vi "OverlayCross.vi"(4 "Color":u32(colorbox)=16711680, 6 "Angle":dbl, 7 "GroupName":string, 8 "error in":errorcluster, 9 "Size":i32=10, 10 "Point":T1, 11 "Image Reference In":T2) -> (0 "error out":errorcluster, 3 "Image Reference Out":T2)   [LabVIEW 2020, in "OpenLvVision_Overlays.lvlib"]
doc: "Overlay a arc on top of an image."
uses:
  OpenLvVision_Overlays.lvlib
  <vilib>/OpenLvVision/OpenLvVision_Image/Management/TypeDef/OLV Image.ctl
  TypeDefs/PointI32.ctl
  <vilib>/OpenLvVision/OpenLvVision_Image/Management/OLV Management.lvlib
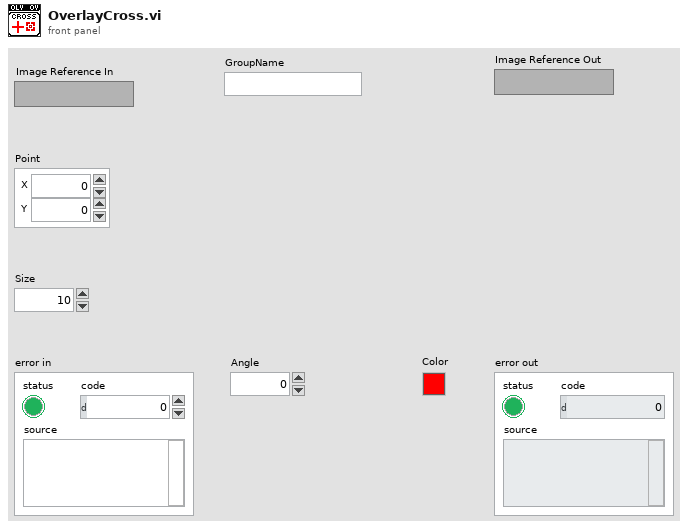
[diagram p1: front panel]
types:
  T1 = typedef "OpenLvVision_Overlays.lvlib/PointI32.ctl" = cluster{"X":i32, "Y":i32}
  T2 = typedef "OLV OpenLvVision_Image.lvlib/OLV Management.lvlib/OLV Image.ctl" = refnum<image>
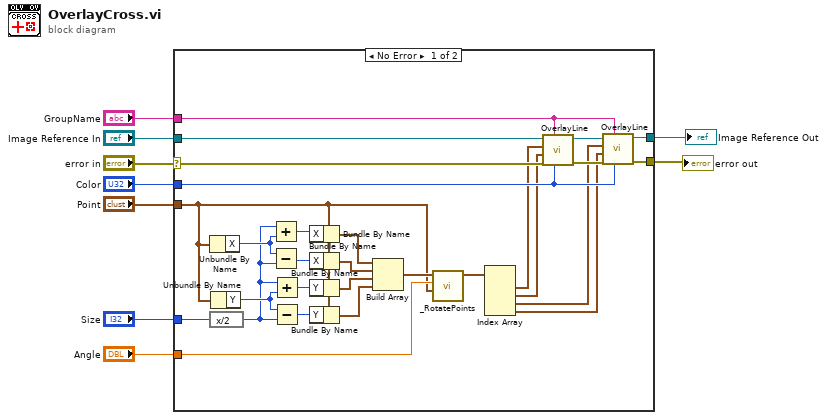
[diagram p0: block diagram]
diagram:
  n1 = case shown="No Error" "error in" {
    selector: "error in" -> [w31 w38]
    tunnel: [w36 w38] -> w8
    tunnel: "Image Reference In" -> [w32 w39]
    tunnel: [w37 w39] -> w7
    tunnel: "GroupName" -> [w33 _]
    tunnel: "Color" -> [w30 _]
    tunnel: "Point" -> [w15 _]
    tunnel: "Size" -> [w23 _]
    tunnel: "Angle" -> [w16 _]
    frame No Error {
      n2 = Unbundle By Name(w15) -> ("X"=w24:i32)
      n3 = expression code="x/2"(w23) -> (w22:i32)
      n4 = Unbundle By Name(w15) -> ("Y"=w27:i32)
      n5 = Add(x=w22, y=w24) -> (x+y=w26:i32)
      n6 = Subtract(x=w24, y=w22) -> (x-y=w25:i32)
      n7 = Add(x=w22, y=w27) -> (x+y=w29:i32)
      n8 = Subtract(x=w27, y=w22) -> (x-y=w28:i32)
      n9 = Bundle By Name(cluster=w15, "X"=w26) -> (w19:T1)
      n10 = Bundle By Name(cluster=w15, "X"=w25) -> (w21:T1)
      n11 = Bundle By Name(cluster=w15, "Y"=w29) -> (w20:T1)
      n12 = Bundle By Name(cluster=w15, "Y"=w28) -> (w18:T1)
      n13 = Build Array(w19, w21, w20, w18) -> (w17:T1[])
      n14 = call "_RotatePoints.vi"("Origin"=w15, "Angle"=w16, "Points in"=w17) -> ("Points out"=w14:T1[])  [unwired: 8 in]
      n15 = Index Array(array=w14) -> (element #1=w13:T1, element #2=w12:T1, element #3=w11:T1, element #4=w10:T1)  [unwired: 4 in]
      n16 = call "OverlayLine.vi"("Color"=w30, "GroupName"=w33, "error in"=w31, "EndPoint"=w12, "StartPoint"=w13, "Image Reference In"=w32) -> ("error out"=w35:errorcluster, "Image Reference Out"=w34:T2)  [unwired: 4 in]
      n17 = call "OverlayLine.vi"("Color"=w30, "GroupName"=w33, "error in"=w35, "EndPoint"=w10, "StartPoint"=w11, "Image Reference In"=w34) -> ("error out"=w36:errorcluster, "Image Reference Out"=w37:T2)  [unwired: 4 in]
    }
    frame Error {
    }
  }
  "error out" <- w8
  "Image Reference Out" <- w7
